vi "Check Return Error.vi"(8 "error in (no error)":errorcluster, 10 "Return code":i32, 11 "Error number":i32) -> (0 "error out":errorcluster)   [LabVIEW 2020, in "wiringPi.lvlib"]
uses:
  wiringPi.lvlib
panel:
  out "Map":map{i32, string}(c390)={25021="Error %d opening SPI device", 25022="Error %d transfering data to/from SPI device", 25023="Error %d closing SPI device", 25031="Error %d opening I2C device", 25032="Error %d reading from I2C device", 25033="Error %d writing to I2C device", 25034="Error %d closing I2C device"}
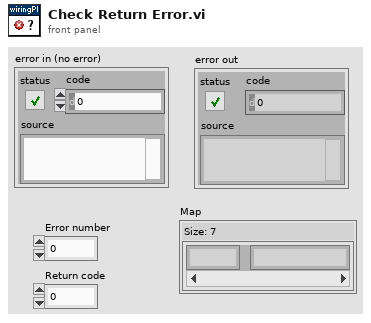
[diagram p1: front panel]
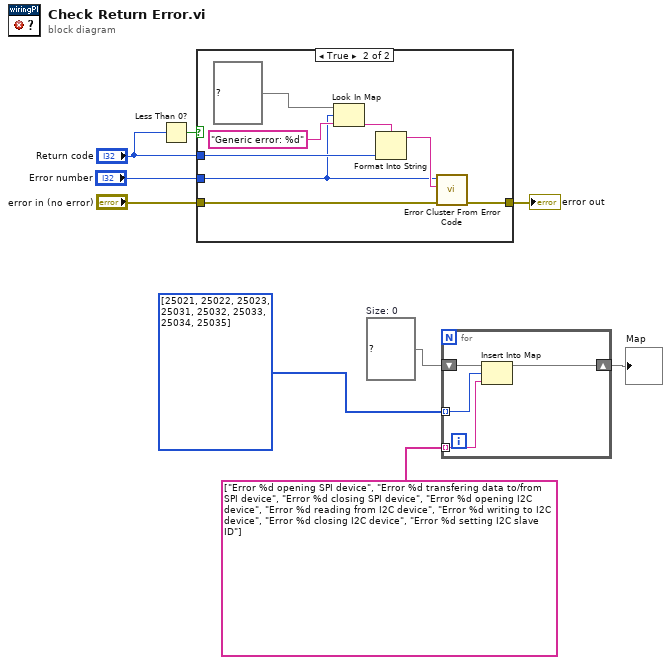
[diagram p0: block diagram]
diagram:
  w3 = map{i32, string} {}  # Size: 0
  n1 = Less Than 0?(x="Return code") -> (x < 0?=w7:bool)
  n2 = case shown="True" w7 {
    tunnel: "error in (no error)" -> [w10 w18]
    tunnel: [w10 w17] -> w9
    tunnel: "Return code" -> [_ w15]
    tunnel: "Error number" -> [_ w12]
    frame False {
    }
    frame True {
      n3 = Look In Map(map=map{i32, string} {25021="Error %d opening SPI device", 25022="Error %d transfering data to/from SPI device", 25023="Error %d closing SPI device", 25031="Error %d opening I2C device", 25032="Error %d reading from I2C device", 25033="Error %d writing to I2C device", 25034="Error %d closing I2C device"} ("Map"), key=w12, default value="Generic error: %d") -> (value=w16:string)  [unwired: 1 out]
      n4 = Format Into String(format string=w16, w15) -> (resulting string=w14:string)  [unwired: 2 in, 1 out]
      n5 = call <vilib>:"Error Cluster From Error Code.vi"("error in (no error)"=w18, "error message (\"\")"=w14, "error code (0)"=w12) -> ("error out"=w17:errorcluster)  [unwired: 6 in]
    }
  }
  "error out" <- w9
  n6 = for {
    tunnel: i32[] [25021, 25022, 25023, 25031, 25032, 25033, 25034, 25035] -> [w21] mode=indexing
    tunnel: string[] ["Error %d opening SPI device", "Error %d transfering data to/from SPI device", "Error %d closing SPI device", "Error %d opening I2C device", "Error %d reading from I2C device", "Error %d writing to I2C device", "Error %d closing I2C device", "Error %d setting I2C slave ID"] -> [w20] mode=indexing
    shift-right: [w19] -> w2
    shift-left: w3 -> [w22]
    n7 = Insert Into Map(map in=w22, key=w21, value=w20) -> (map out=w19:map{i32, string})  [unwired: 2 out]
  }
  "Map" <- w2
